vi "write final cache to tdms.vi"(0 "tdms file in":refnum<k34>, 1 "sample counter":i32, 5 "cache in":T2, 7 "dictionary group names":T1, 9 "output type order":T3[](array[typedef]), 11 "error in":errorcluster, 12 "scans per write":u16=20, 13 "dictionary":T1) -> (6 "cache out":T2, 15 "error out":errorcluster)   [LabVIEW 2015, in "TDMS datalogger runtime.lvclass"]
uses:
  TDMS datalogger runtime.lvclass
  <vilib>/NI/Tag Bus/tag/Data Type.ctl
  data cache.ctl
  <vilib>/NI/Tag Bus/dictionary/full data dictionary.ctl
  <vilib>/NI/Tag Bus/tag/tag descriptor.lvclass
  <vilib>/NI/Tag Bus/dictionary/data dictionary.lvclass
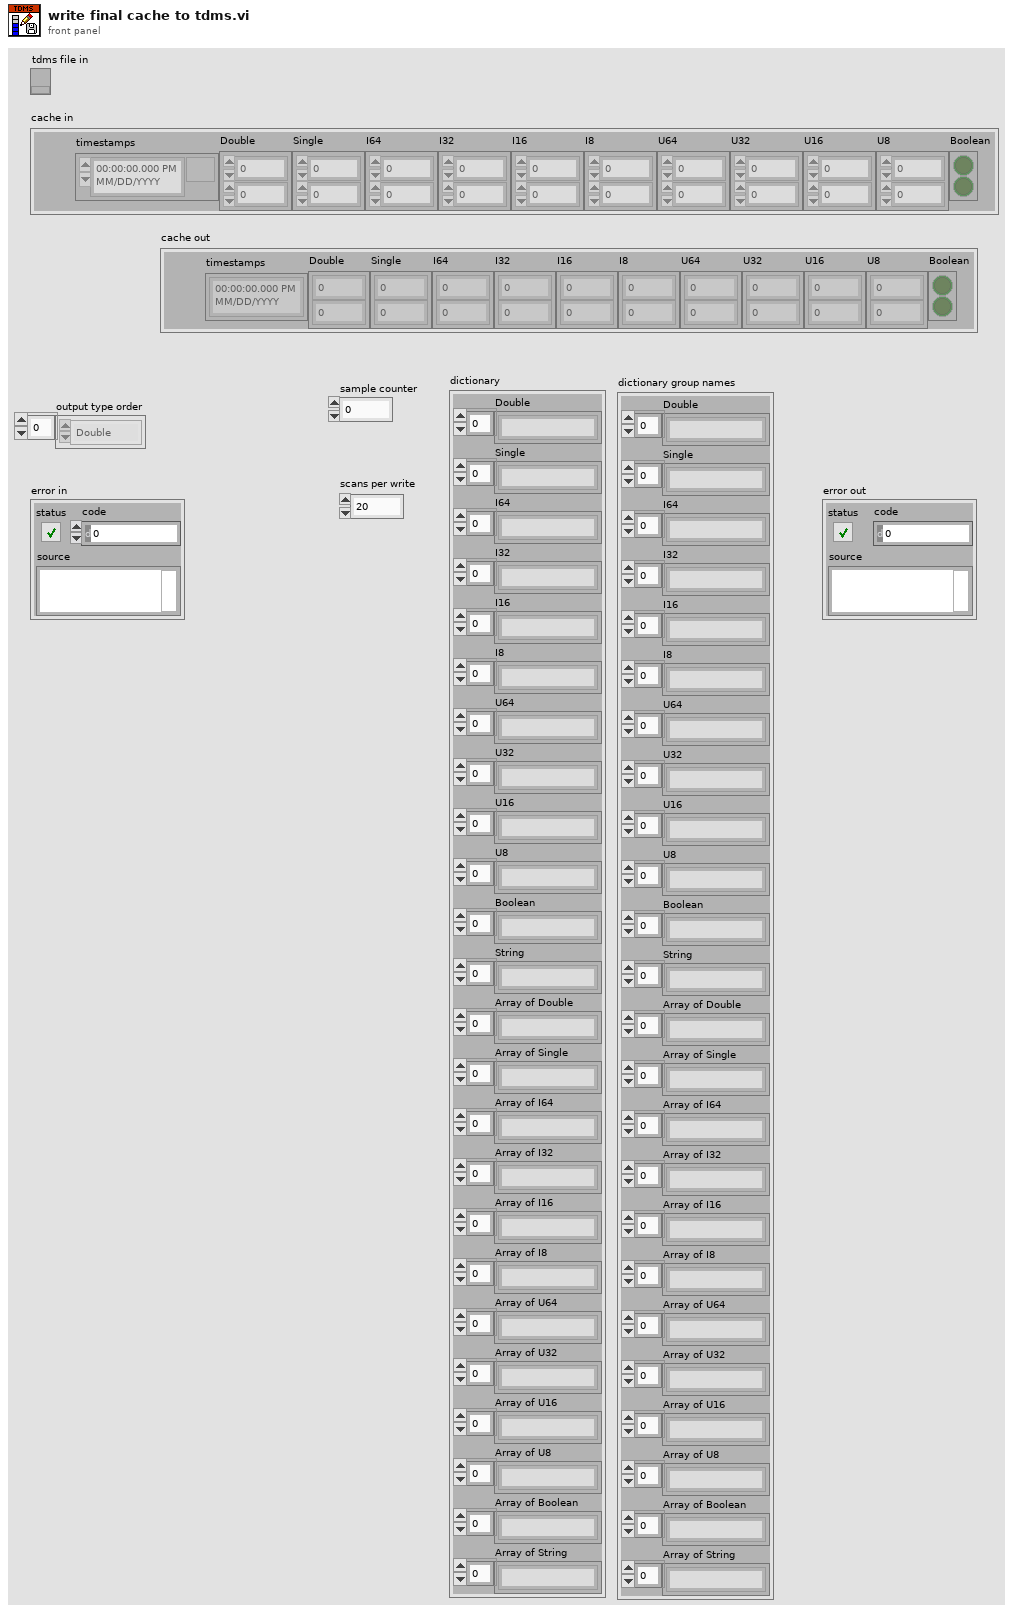
[diagram p1: front panel]
types:
  T1 = typedef "tag bus.lvlib/data dictionary.lvclass/full data dictionary.ctl" = cluster{"Double":string[], "Single":string[], "I64":string[], "I32":string[], "I16":string[], "I8":string[], "U64":string[], "U32":string[], "U16":string[], "U8":string[], "Boolean":string[], "String":string[], "Array of Double":string[], "Array of Single":string[], "Array of I64":string[], "Array of I32":string[], "Array of I16":string[], "Array of I8":string[], "Array of U64":string[], "Array of U32":string[], "Array of U16":string[], "Array of U8":string[], "Array of Boolean":string[], "Array of String":string[]}
  T2 = typedef "TDMS datalogger runtime.lvclass/data cache.ctl" = cluster{"timestamps":timestamp[], "Double":dbl[][], "Single":sgl[][], "I64":i64[][], "I32":i32[][], "I16":i16[][], "I8":i8[][], "U64":u64[][], "U32":u32[][], "U16":u16[][], "U8":u8[][], "Boolean":bool[][]}
  T3 = typedef "tag bus.lvlib/tag descriptor.lvclass/Data Type.ctl" = enum16{"Double", "Single", "I64", "I32", "I16", "I8", "U64", "U32", "U16", "U8", "Boolean", "String", "Array of Double", "Array of Single", "Array of I64", "Array of I32", "Array of I16", "Array of I8", "Array of U64", "Array of U32", "Array of U16", "Array of U8", "Array of Boolean", "Array of String"}
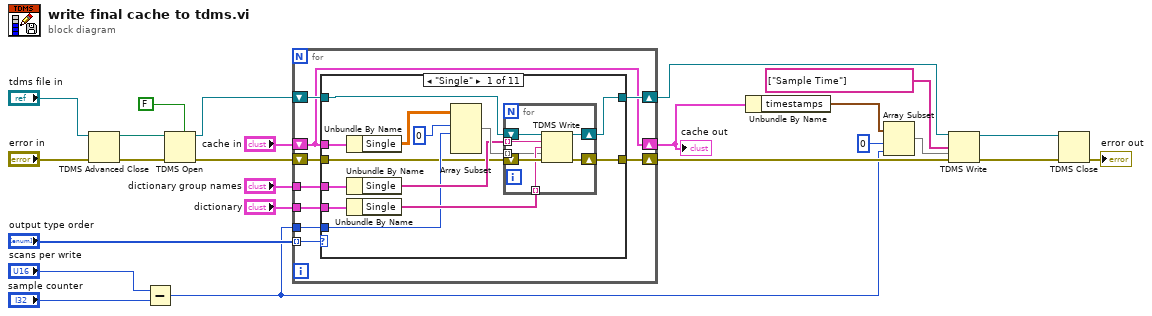
[diagram p0: block diagram]
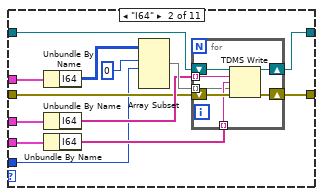
[diagram p2: hidden frame]
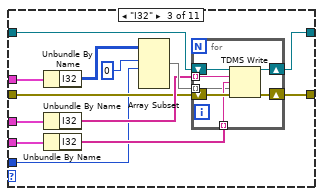
[diagram p3: hidden frame]
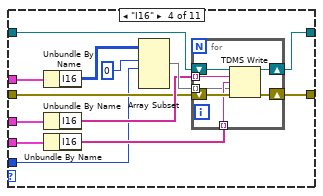
[diagram p4: hidden frame]
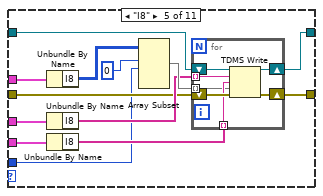
[diagram p5: hidden frame]
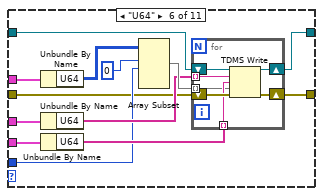
[diagram p6: hidden frame]
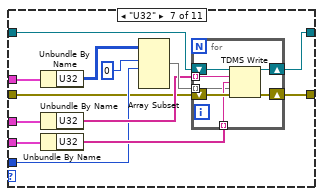
[diagram p7: hidden frame]
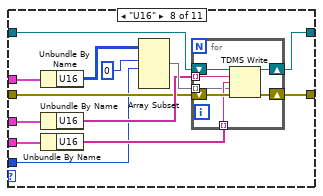
[diagram p8: hidden frame]
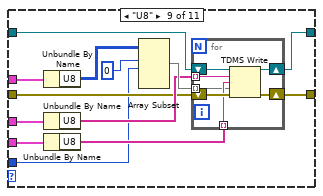
[diagram p9: hidden frame]
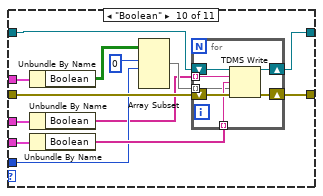
[diagram p10: hidden frame]
diagram:
  n1 = TDMS Advanced Close(8:"error in", 11:"tdms file in") -> (0:w19:errorcluster, 3:w18:path)  [unwired: 2 in]
  n2 = Subtract(x="scans per write", y="sample counter") -> (x-y=w7:i32)
  n3 = TDMS Open(5:FALSE ("create index file? (T)"), 8:w19, 11:w18) -> (0:w15:errorcluster, 3:w16:refnum<k34>)  [unwired: 4 in]
  n4 = for {
    tunnel: "output type order" -> [w30] mode=indexing
    shift-right: [w31] -> w14
    shift-left: w15 -> [w32]
    shift-right: [w29] -> w13
    shift-left: w16 -> [w33]
    shift-right: [w28] -> w22
    shift-left: "cache in" -> [w28]
    tunnel: "dictionary" -> [w27]
    tunnel: "dictionary group names" -> [w26]
    tunnel: w7 -> [w25]
    n5 = case shown="\"Single\"" w30 {
      tunnel: w33 -> [w40 w59 w75 w99 w116 w139 w159 w179 w199 w221 w234]
      tunnel: w32 -> [w34 w58 w76 w97 w115 w134 w155 w177 w197 w224 w235]
      tunnel: [w42 w61 w80 w101 w121 w141 w161 w181 w201 w223 w235] -> w31
      tunnel: w28 -> [w39 w57 w81 w98 w119 w138 w154 w178 w198 w226 _]
      tunnel: [w41 w60 w79 w100 w120 w140 w160 w180 w200 w222 w234] -> w29
      tunnel: w27 -> [w37 w55 w78 w96 w117 w136 w157 w176 w194 w225 _]
      tunnel: w26 -> [w38 w56 w77 w95 w118 w137 w156 w175 w195 w215 _]
      tunnel: w25 -> [w36 w54 w74 w94 w114 w135 w158 w174 w196 w217 _]
      frame "Single" {
        n6 = Unbundle By Name(w39) -> ("Single"=w35:sgl[][])
        n7 = Unbundle By Name(w38) -> ("Single"=w43:string[])
        n8 = Unbundle By Name(w37) -> ("Single"=w46:string[])
        n9 = Array Subset(array=w35, index (row)=0 ("index"), length (row)=w36) -> (w44:sgl[][])  [unwired: 2 in]
        n10 = for {
          tunnel: w46 -> [w49] mode=indexing
          tunnel: w44 -> [w48] mode=indexing
          tunnel: w43 -> [w47] mode=indexing
          shift-right: [w52] -> w42
          shift-left: w34 -> [w53]
          shift-right: [w51] -> w41
          shift-left: w40 -> [w50]
          n11 = TDMS Write(0:w50, 5:w47, 7:w49, 9:w48, 11:w53) -> (4:w51:refnum<k34>, 15:w52:errorcluster)  [unwired: 1 in, 2 out]
        }
      }
      frame "I64" {
        n12 = Unbundle By Name(w57) -> ("I64"=w66:i64[][])
        n13 = Unbundle By Name(w56) -> ("I64"=w62:string[])
        n14 = Unbundle By Name(w55) -> ("I64"=w65:string[])
        n15 = Array Subset(array=w66, index (row)=0 ("index"), length (row)=w54) -> (w63:i64[][])  [unwired: 2 in]
        n16 = for {
          tunnel: w65 -> [w69] mode=indexing
          tunnel: w63 -> [w68] mode=indexing
          tunnel: w62 -> [w67] mode=indexing
          shift-right: [w72] -> w61
          shift-left: w58 -> [w73]
          shift-right: [w71] -> w60
          shift-left: w59 -> [w70]
          n17 = TDMS Write(0:w70, 5:w67, 7:w69, 9:w68, 11:w73) -> (4:w71:refnum<k34>, 15:w72:errorcluster)  [unwired: 1 in, 2 out]
        }
      }
      frame "I32" {
        n18 = Unbundle By Name(w81) -> ("I32"=w86:i32[][])
        n19 = Unbundle By Name(w77) -> ("I32"=w82:string[])
        n20 = Unbundle By Name(w78) -> ("I32"=w85:string[])
        n21 = Array Subset(array=w86, index (row)=0 ("index"), length (row)=w74) -> (w83:i32[][])  [unwired: 2 in]
        n22 = for {
          tunnel: w85 -> [w89] mode=indexing
          tunnel: w83 -> [w88] mode=indexing
          tunnel: w82 -> [w87] mode=indexing
          shift-right: [w92] -> w80
          shift-left: w76 -> [w93]
          shift-right: [w91] -> w79
          shift-left: w75 -> [w90]
          n23 = TDMS Write(0:w90, 5:w87, 7:w89, 9:w88, 11:w93) -> (4:w91:refnum<k34>, 15:w92:errorcluster)  [unwired: 1 in, 2 out]
        }
      }
      frame "I16" {
        n24 = Unbundle By Name(w98) -> ("I16"=w106:i16[][])
        n25 = Unbundle By Name(w95) -> ("I16"=w102:string[])
        n26 = Unbundle By Name(w96) -> ("I16"=w105:string[])
        n27 = Array Subset(array=w106, index (row)=0 ("index"), length (row)=w94) -> (w103:i16[][])  [unwired: 2 in]
        n28 = for {
          tunnel: w105 -> [w109] mode=indexing
          tunnel: w103 -> [w108] mode=indexing
          tunnel: w102 -> [w107] mode=indexing
          shift-right: [w112] -> w101
          shift-left: w97 -> [w113]
          shift-right: [w111] -> w100
          shift-left: w99 -> [w110]
          n29 = TDMS Write(0:w110, 5:w107, 7:w109, 9:w108, 11:w113) -> (4:w111:refnum<k34>, 15:w112:errorcluster)  [unwired: 1 in, 2 out]
        }
      }
      frame "I8" {
        n30 = Unbundle By Name(w119) -> ("I8"=w126:i8[][])
        n31 = Unbundle By Name(w118) -> ("I8"=w122:string[])
        n32 = Unbundle By Name(w117) -> ("I8"=w125:string[])
        n33 = Array Subset(array=w126, index (row)=0 ("index"), length (row)=w114) -> (w123:i8[][])  [unwired: 2 in]
        n34 = for {
          tunnel: w125 -> [w129] mode=indexing
          tunnel: w123 -> [w128] mode=indexing
          tunnel: w122 -> [w127] mode=indexing
          shift-right: [w132] -> w121
          shift-left: w115 -> [w133]
          shift-right: [w131] -> w120
          shift-left: w116 -> [w130]
          n35 = TDMS Write(0:w130, 5:w127, 7:w129, 9:w128, 11:w133) -> (4:w131:refnum<k34>, 15:w132:errorcluster)  [unwired: 1 in, 2 out]
        }
      }
      frame "U64" {
        n36 = Unbundle By Name(w138) -> ("U64"=w146:u64[][])
        n37 = Unbundle By Name(w137) -> ("U64"=w142:string[])
        n38 = Unbundle By Name(w136) -> ("U64"=w145:string[])
        n39 = Array Subset(array=w146, index (row)=0 ("index"), length (row)=w135) -> (w143:u64[][])  [unwired: 2 in]
        n40 = for {
          tunnel: w145 -> [w149] mode=indexing
          tunnel: w143 -> [w148] mode=indexing
          tunnel: w142 -> [w147] mode=indexing
          shift-right: [w152] -> w141
          shift-left: w134 -> [w153]
          shift-right: [w151] -> w140
          shift-left: w139 -> [w150]
          n41 = TDMS Write(0:w150, 5:w147, 7:w149, 9:w148, 11:w153) -> (4:w151:refnum<k34>, 15:w152:errorcluster)  [unwired: 1 in, 2 out]
        }
      }
      frame "U32" {
        n42 = Unbundle By Name(w154) -> ("U32"=w166:u32[][])
        n43 = Unbundle By Name(w156) -> ("U32"=w162:string[])
        n44 = Unbundle By Name(w157) -> ("U32"=w165:string[])
        n45 = Array Subset(array=w166, index (row)=0 ("index"), length (row)=w158) -> (w163:u32[][])  [unwired: 2 in]
        n46 = for {
          tunnel: w165 -> [w169] mode=indexing
          tunnel: w163 -> [w168] mode=indexing
          tunnel: w162 -> [w167] mode=indexing
          shift-right: [w172] -> w161
          shift-left: w155 -> [w173]
          shift-right: [w171] -> w160
          shift-left: w159 -> [w170]
          n47 = TDMS Write(0:w170, 5:w167, 7:w169, 9:w168, 11:w173) -> (4:w171:refnum<k34>, 15:w172:errorcluster)  [unwired: 1 in, 2 out]
        }
      }
      frame "U16" {
        n48 = Unbundle By Name(w178) -> ("U16"=w186:u16[][])
        n49 = Unbundle By Name(w175) -> ("U16"=w182:string[])
        n50 = Unbundle By Name(w176) -> ("U16"=w185:string[])
        n51 = Array Subset(array=w186, index (row)=0 ("index"), length (row)=w174) -> (w183:u16[][])  [unwired: 2 in]
        n52 = for {
          tunnel: w185 -> [w189] mode=indexing
          tunnel: w183 -> [w188] mode=indexing
          tunnel: w182 -> [w187] mode=indexing
          shift-right: [w192] -> w181
          shift-left: w177 -> [w193]
          shift-right: [w191] -> w180
          shift-left: w179 -> [w190]
          n53 = TDMS Write(0:w190, 5:w187, 7:w189, 9:w188, 11:w193) -> (4:w191:refnum<k34>, 15:w192:errorcluster)  [unwired: 1 in, 2 out]
        }
      }
      frame "U8" {
        n54 = Unbundle By Name(w198) -> ("U8"=w206:u8[][])
        n55 = Unbundle By Name(w195) -> ("U8"=w202:string[])
        n56 = Unbundle By Name(w194) -> ("U8"=w205:string[])
        n57 = Array Subset(array=w206, index (row)=0 ("index"), length (row)=w196) -> (w203:u8[][])  [unwired: 2 in]
        n58 = for {
          tunnel: w205 -> [w209] mode=indexing
          tunnel: w203 -> [w208] mode=indexing
          tunnel: w202 -> [w207] mode=indexing
          shift-right: [w212] -> w201
          shift-left: w197 -> [w213]
          shift-right: [w211] -> w200
          shift-left: w199 -> [w210]
          n59 = TDMS Write(0:w210, 5:w207, 7:w209, 9:w208, 11:w213) -> (4:w211:refnum<k34>, 15:w212:errorcluster)  [unwired: 1 in, 2 out]
        }
      }
      frame "Boolean" {
        n60 = Unbundle By Name(w226) -> ("Boolean"=w219:bool[][])
        n61 = Unbundle By Name(w215) -> ("Boolean"=w214:string[])
        n62 = Unbundle By Name(w225) -> ("Boolean"=w220:string[])
        n63 = Array Subset(array=w219, index (row)=0 ("index"), length (row)=w217) -> (w216:bool[][])  [unwired: 2 in]
        n64 = for {
          tunnel: w220 -> [w229] mode=indexing
          tunnel: w216 -> [w228] mode=indexing
          tunnel: w214 -> [w227] mode=indexing
          shift-right: [w232] -> w223
          shift-left: w224 -> [w233]
          shift-right: [w231] -> w222
          shift-left: w221 -> [w230]
          n65 = TDMS Write(0:w230, 5:w227, 7:w229, 9:w228, 11:w233) -> (4:w231:refnum<k34>, 15:w232:errorcluster)  [unwired: 1 in, 2 out]
        }
      }
      frame Default {
      }
    }
  }
  "cache out" <- w22
  n66 = Unbundle By Name(w22) -> ("timestamps"=w6:timestamp[])
  n67 = Array Subset(array=w6, index=0, length=w7) -> (w5:timestamp[])
  n68 = TDMS Write(0:w13, 7:string[] ["Sample Time"] ("channel name(s)"), 9:w5, 11:w14) -> (4:w2:refnum<k34>, 15:w4:errorcluster)  [unwired: 2 in, 2 out]
  n69 = TDMS Close(8:w4, 11:w2) -> (0:→"error out":errorcluster)  [unwired: 1 out]
